vi "consumer.vi"() -> ()   [LabVIEW 2020]
uses:
  <userlib>/Zaphiro/GTools/Redis/Sources/Redis/Redis.lvclass/Redis.ctl
  aea59807-97c7-47ab-b578-198c3bfad1a9.vi
  f854457d-36a3-4227-beff-9843280818cc.vi
  b567c38f-e722-4316-83bf-2d80707c7bfa.vi
  <userlib>/Zaphiro/GTools/Redis/Sources/Redis/Connection/PING.vi
  aea59807-97c7-47ab-b578-198c3bfad1a9.vi/7c7783df-fd5a-49d9-9b7a-63cc9fb0e4e5.vi
  <userlib>/Zaphiro/GTools/Redis/Sources/Redis/Connection/QUIT.vi
  <userlib>/Zaphiro/GTools/Redis/Sources/Redis/subVIs/LL_collect-response.vi
  <userlib>/Zaphiro/GTools/Redis/Sources/Redis/Redis.lvclass
  <vilib>/Comparison/Less/Less Functor/Less Functor.lvclass
panel:
  in  "lb-meas":i32[](listbox) caption="Available measurements"
  out "values":string[](array[string])
  out "measurements":string[](array[string])
  in  "lb-ts":i32(listbox) caption="Available HASH (timestamps)"
  in  "check-ts":bool
  in  "check-list":bool
  in  "connection":cluster{"ip":string, "port":u16, "timeout":i32}={"ip"="localhost", "port"=6379, "timeout"=1000}
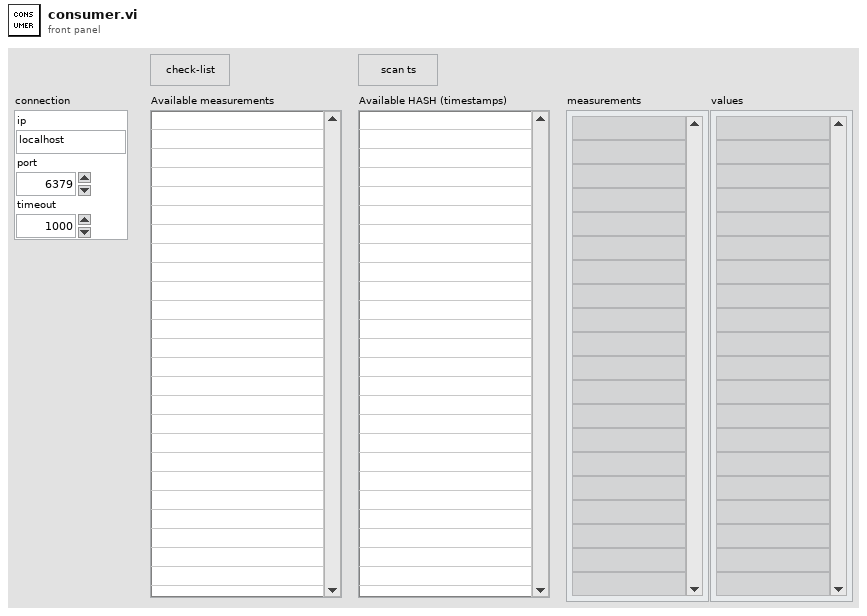
[diagram p1: front panel]
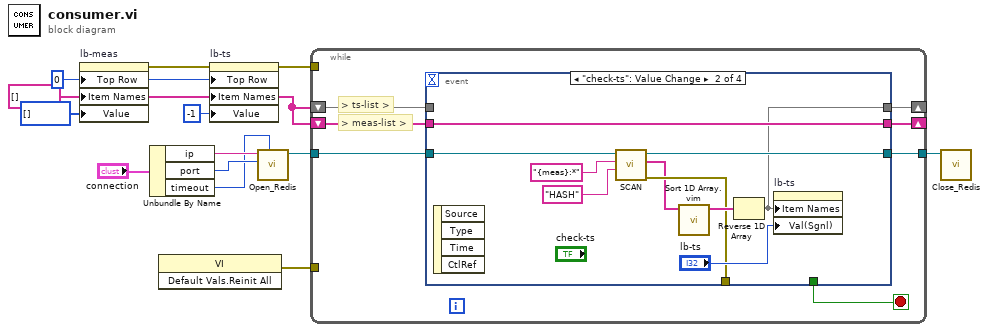
[diagram p0: block diagram]
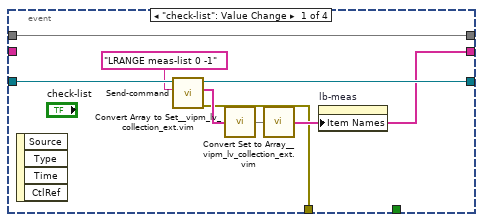
[diagram p2: hidden frame]
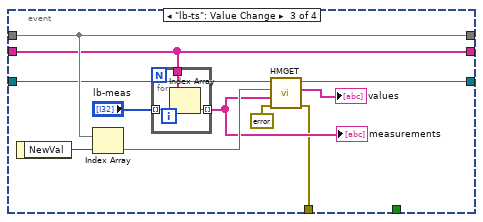
[diagram p3: hidden frame]
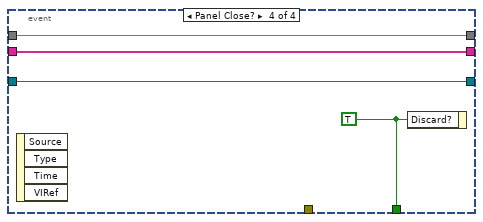
[diagram p4: hidden frame]
diagram:
  w1 = 0 ("Top Row")
  w3 = string[] [] ("Item Names")
  n1 = property on="lb-meas" class="LstBox (strict)"("Top Row"=w1, "Item Names"=w3, "Value"=i32[] [] ("lb-meas")) -> (error out=w4:errorcluster)  [unwired: 2 in, 1 out]
  n2 = Unbundle By Name("connection") -> ("ip"=w12:string, "port"=w11:u16, "timeout"=w10:i32)
  n3 = invoke class="VI" method="Default Vals.Reinit All"() -> (error out=w2:errorcluster)  [unwired: 3 in, 2 out]
  n4 = property on="lb-ts" class="LstBox (strict)"(error in=w4, "Top Row"=w1, "Item Names"=w3, "Value"=-1 ("available timestamps")) -> (error out=w7:errorcluster)  [unwired: 1 in, 1 out]
  n5 = call <userlib>:"Open_Redis.vi"("Tcp timeout ms"=w10, "Port"=w11, "Host"=w12) -> ("output cluster"=w9:refnum<class "Redis.lvclass">)  [unwired: 6 in, 2 out]
  n6 = while {
    tunnel: w9 -> [w20]
    tunnel: [w19] -> w8
    shift-right: [w17] -> _
    shift-left: w3 -> [w16]
    shift-right: [w15] -> _
    shift-left: w3 -> [w14]
    tunnel: w7 -> [_]
    tunnel: w2 -> [_]
    stop <- w18 stop-if-true
    # "> ts-list >"
    # "> meas-list >"
    n7 = event shown="[1] \"check-ts\": Value Change" {
      selector: _ -> [_ _ _ _]
      dyn-events: _ -> [_ _ _ _]
      timeout: _ -> [_ _ _ _]
      tunnel: w20 -> [w28 w37 w47 w55]
      tunnel: [w27 w36 w48 w55] -> w19
      tunnel: [_ _ _ w56] -> w18
      tunnel: [w22 w38 w41 w54] -> w17
      tunnel: w16 -> [_ w38 w41 w54]
      tunnel: [w23 w29 w49 w53] -> w15
      tunnel: w14 -> [w23 _ w49 w53]
      tunnel: [w21 w31 w39 _] -> _
      event "check-list": Value Change {
        n8 = event-data() -> ()  [unwired: 1 in, 4 out]
        n9 = call <userlib>:"Send-command.vi"("command"="LRANGE meas-list 0 -1" ("Key"), "Redis.lvclass in"=w28) -> ("error out"=w21:errorcluster, "redis reply"=w24:string[], "Redis.lvclass out"=w27:refnum<class "Redis.lvclass">)  [unwired: 7 in]
        n10 = call "Convert Array to Set__vipm_lv_collection_ext.vim"("array"=w24) -> ("set"=w25:set{string})  [unwired: 6 in]
        n11 = call "Convert Set to Array__vipm_lv_collection_ext.vim"("set"=w25) -> ("array"=w22:string[])  [unwired: 8 in]
        n12 = property on="lb-meas" class="LstBox (strict)"("Item Names"=w22) -> ()  [unwired: 2 in, 2 out]
      }
      event "check-ts": Value Change {
        n13 = event-data() -> ()  [unwired: 1 in, 4 out]
        n14 = call <userlib>:"SCAN.vi"("Type"="HASH" ("Key"), "Pattern"="{meas}:*" ("Key"), "Redis.lvclass in"=w37) -> ("error out"=w31:errorcluster, "redis reply"=w30:string[], "Redis.lvclass out"=w36:refnum<class "Redis.lvclass">)  [unwired: 6 in]
        n15 = call "Sort 1D Array.vim"("unsorted array"=w30) -> ("sorted array"=w33:string[])  [unwired: 10 in]
        n16 = Reverse 1D Array(array=w33) -> (reversed array=w29:string[])
        n17 = property on="lb-ts" class="LstBox (strict)"("Item Names"=w29, "Val(Sgnl)"="lb-ts") -> ()  [unwired: 2 in, 2 out]
      }
      event "lb-ts": Value Change {
        n18 = event-data() -> ("NewVal"=w43:i32)  [unwired: 1 in]
        n19 = Index Array(array=w49, index=w43) -> (element=w46:string)
        n20 = for {
          tunnel: "lb-meas" -> [w51] mode=indexing
          tunnel: w41 -> [w52]
          tunnel: [w50] -> w40 mode=indexing
          n21 = Index Array(array=w52, index=w51) -> (element=w50:string)
        }
        "measurements" <- w40
        n22 = call <userlib>:"HMGET.vi"("error in"=errorcluster {"status"=FALSE, "code"=0, "source"=""}, "Fields"=w40, "Key"=w46, "Redis.lvclass in"=w47) -> ("error out"=w39:errorcluster, "redis reply"=→"values":string[], "Redis.lvclass out"=w48:refnum<class "Redis.lvclass">)  [unwired: 5 in]
      }
      event Panel Close? {
        w56 = TRUE ("Discard?")
        n23 = event-data() -> ()  [unwired: 1 in, 4 out]
        n24 = event-data("Discard?"=w56) -> ()  [unwired: 1 in, 1 out]
      }
    }
  }
  n25 = call <userlib>:"Close_Redis.vi"("Redis.lvclass in"=w8) -> ()  [unwired: 9 in, 2 out]
